vi "variant to path.vi"(1 "Variant":variant) -> (0 "Path":path)   [LabVIEW 2025]
doc: "convert variant data to a LabVIEW String\n<B>Input:</B>\nVariant (skalar)\n<B>Output:</B>\nString"
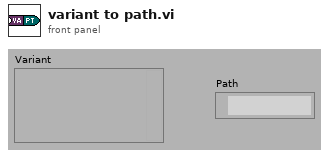
[diagram p1: front panel]
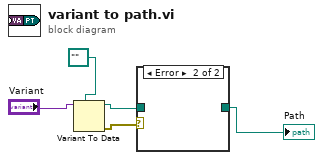
[diagram p0: block diagram]
diagram:
  n1 = Variant To Data(type=path "", Variant="Variant") -> (data=w4:path, error out=w3:errorcluster)  [unwired: 1 in]
  n2 = case shown="Error" w3 {
    tunnel: w4 -> [w6 _]
    tunnel: [w6 _] -> w1
    frame No Error {
    }
    frame Error {
    }
  }
  "Path" <- w1
